vi "Create.vi"(7 "Direction":T1, 8 "error in (no error)":errorcluster, 9 "Custom Config Data":u8[](array[numeric]), 10 "Name":string, 11 "CIFFIFO in":refnum<class "CIF_Iceoryx_PCAP_Universal.lvclass">) -> (0 "error out":errorcluster, 3 "CIFFIFO out":refnum<class "CIF_Iceoryx_PCAP_Universal.lvclass">)   [LabVIEW 2021, in "CIF_Iceoryx_PCAP_Universal.lvclass"]
uses:
  CIF_Iceoryx_PCAP_Universal.lvclass
  ChannelCommon/typedef/Direction.ctl
  D:/dev/Packages/CIF_Channels_Core/src/CIFChannels/CIFChannels.lvclass
  <vilib>/CIF Foundation/CIF Utilities/Statistics/I64/Stats_I64_CIF_U.lvclass/Stats_I64_CIF_U.ctl
  ChannelCommon/typedef/Channel State.ctl
  ChannelCommon/typedef/Channel Pattern.ctl
  ChannelCommon/typedef/Disconnect Behavior.ctl
  CIFChannels/CIFChannels.lvclass/CIFChannels.ctl
  CIF_Iceoryx_PCAP_Universal.lvclass/CIF_Iceoryx_PCAP_Universal.ctl
  CIFChannels/Accessors/Write Channel State.vi
  CIFChannels/Accessors/Write Subscriber Count.vi
  CIFChannels/Accessors/Write Pattern.vi
  CIFChannels/Accessors/Write Channel Benchmark.vi
  CIFChannels/Accessors/Write Flatten Benchmark.vi
  CIFChannels/Accessors/Write Channel Class.vi
  <vilib>/CIF Foundation/CIF Utilities/Statistics/I64/Stats_I64_CIF_U.lvclass
  CIFChannels/CIFChannels.lvclass
  ChannelCommon/ChannelCommon.lvlib
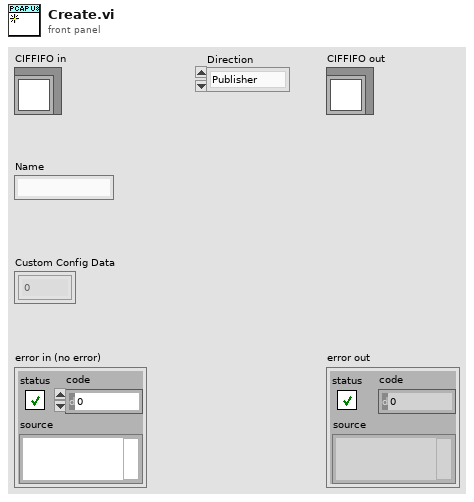
[diagram p1: front panel]
types:
  T1 = typedef "ChannelCommon.lvlib/Direction.ctl" = enum8{"Publisher", "Subscriber"}
  T2 = typedef "ChannelCommon.lvlib/Channel State.ctl" = enum8{"Creating", "Disconnected", "Connecting", "Connected", "Destroyed"}
  T3 = typedef "ChannelCommon.lvlib/Channel Pattern.ctl" = enum8{"Unknown", "Tag", "FIFO", "MultiFIFO", "BackpressureFIFO"}
  T4 = typedef "ChannelCommon.lvlib/Disconnect Behavior.ctl" = enum8{"Default value", "Last value", "Error with default"}
  T5 = typedef "CIF_Iceoryx_PCAP_Universal.lvclass/FIFO Configuration.ctl" = cluster{"Max Bytes":u32, "Best Effort Queue Depth":u32, "Best Effort Subscribers":u32, "Backpressure Queue Depth":u32, "Backpressure Subscribers":u32, "Linktype":u32}
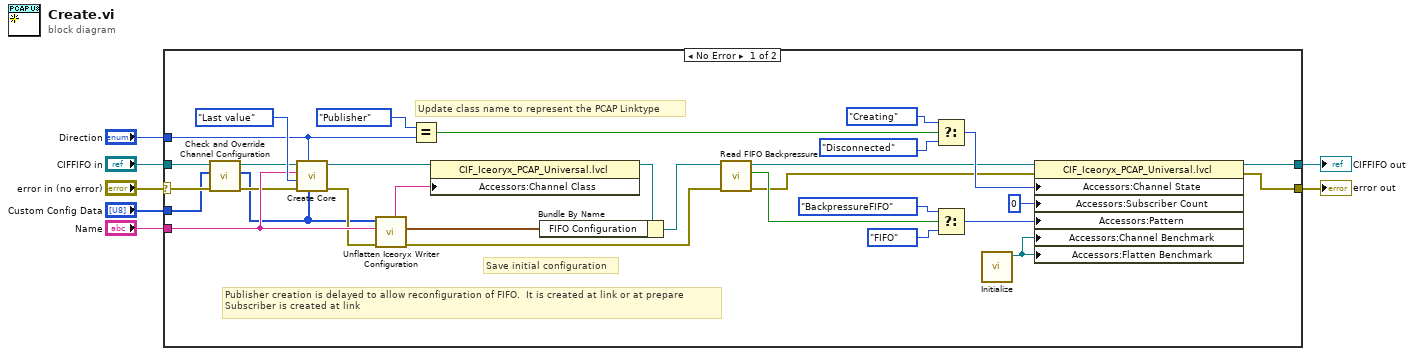
[diagram p0: block diagram]
diagram:
  n1 = case shown="No Error" "error in (no error)" {
    selector: "error in (no error)" -> [w33 w40]
    tunnel: [w14 w40] -> w6
    tunnel: [w35 w39] -> w1
    tunnel: "CIFFIFO in" -> [w34 w39]
    tunnel: "Name" -> [w37 _]
    tunnel: "Direction" -> [w19 _]
    tunnel: "Custom Config Data" -> [w30 _]
    frame No Error {
      # "Save initial configuration"
      # "Update class name to represent the PCAP Linktype"
      # "Publisher creation is delayed to allow reconfiguration of FIFO.  It is created at link or at prepare\nSubscriber is created at link"
      n2 = call-dynamic "Check and Override Channel Configuration.vi"("error in (no error)"=w33, "Custom Config Data in"=w30, "CIFFIFO in"=w34) -> ("error out"=w31:errorcluster, "Custom Config Data out"=w24:u8[], "CIFFIFO out"=w32:refnum<class "CIF_Iceoryx_PCAP_Universal.lvclass">)  [unwired: 6 in]
      n3 = call "Create Core.vi"("Custom Config Data"=w24, "Direction"=w19, "error in (no error)"=w31, "Disconnect Behavior"=Disconnect_Behavior."Last value", "Name"=w37, "CIFChannels in"=w32) -> ("error out"=w36:errorcluster, "CIFChannels out"=w29:refnum<class "CIF_Iceoryx_PCAP_Universal.lvclass">)  [unwired: 1 in, 3 out]
      n4 = call "Unflatten Iceoryx Writer Configuration.vi"("error in"=w36, "Name"=w37, "Custom Config Data in"=w24) -> ("error out"=w9:errorcluster, "FIFO Configuration"=w20:T5, "Updated Class Name"=w22:string)  [unwired: 5 in, 1 out]
      n5 = Equal?(x=Direction."Publisher", y=w19) -> (x = y?=w18:bool)
      n6 = property class="CIF_Iceoryx_PCAP_Universal.lvcl"(reference=w29, "Accessors:Channel Class"=w22) -> (reference out=w21:refnum<class "CIF_Iceoryx_PCAP_Universal.lvclass">)  [unwired: 1 in, 1 out]
      n7 = Bundle By Name(cluster=w21, "FIFO Configuration"=w20) -> (w23:refnum<class "CIF_Iceoryx_PCAP_Universal.lvclass">)
      n8 = call "Read FIFO Backpressure.vi"("error in (no error)"=w9, "CIFChannels in"=w23) -> ("error out"=w8:errorcluster, "Backpressure"=w25:bool, "CIFChannels out"=w10:refnum<class "CIF_Iceoryx_PCAP_Universal.lvclass">)  [unwired: 7 in]
      n9 = Select(t=Channel_State."Creating" ("Channel State"), s=w18, f=Channel_State."Disconnected" ("Channel State")) -> (s? t:f=w15:T2)
      n10 = Select(t=Channel_Pattern."BackpressureFIFO" ("Pattern"), s=w25, f=Channel_Pattern."FIFO" ("Pattern")) -> (s? t:f=w11:T3)
      n11 = call <vilib>:"Initialize.vi"() -> ("Stats_I64_CIF_U out"=w12:refnum<class "Stats_I64_CIF_U.lvclass">)  [unwired: 10 in, 1 out]
      n12 = property class="CIF_Iceoryx_PCAP_Universal.lvcl"(reference=w10, error in=w8, "Accessors:Channel State"=w15, "Accessors:Subscriber Count"=u32 0 ("Subscriber Count"), "Accessors:Pattern"=w11, "Accessors:Channel Benchmark"=w12, "Accessors:Flatten Benchmark"=w12) -> (reference out=w35:refnum<class "CIF_Iceoryx_PCAP_Universal.lvclass">, error out=w14:errorcluster)
    }
    frame Error {
    }
  }
  "error out" <- w6
  "CIFFIFO out" <- w1
